vi "Set Group Privilege.vi"(4 "New Value":bool, 5 "Save File":bool=TRUE, 6 "error in (no error)":errorcluster, 7 "Privilege":string, 8 "Group Name":string, 9 "EasyUserManager in":refnum<class "EasyUserManager.lvclass">) -> (0 "error out":errorcluster, 3 "EasyUserManager out":refnum<class "EasyUserManager.lvclass">)   [LabVIEW 2024, in "EasyUserManager.lvclass"]
doc: "Set <B>Privilege</B> (e.g. Operate.Execute) to the specified <B>New Value</B> for the group called <B>Group Name</B>. \n\nThe boolean input <B>Save File</B> controls whether changes are immediately saved to the users file (Default: True)."
uses:
  EasyUserManager.lvclass
  EasyUserManager.lvclass/EasyUserManager.ctl
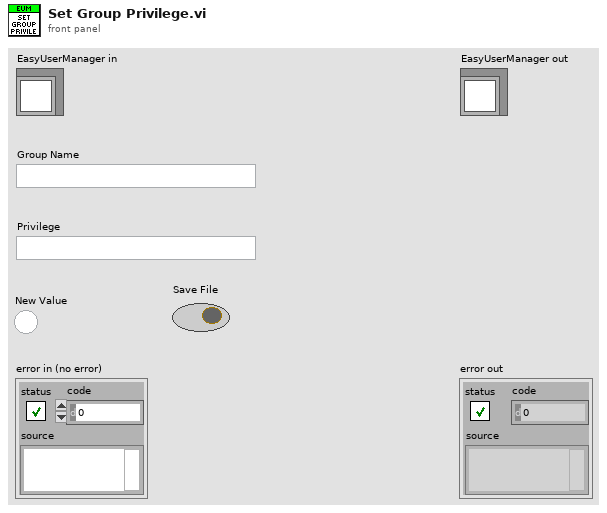
[diagram p1: front panel]
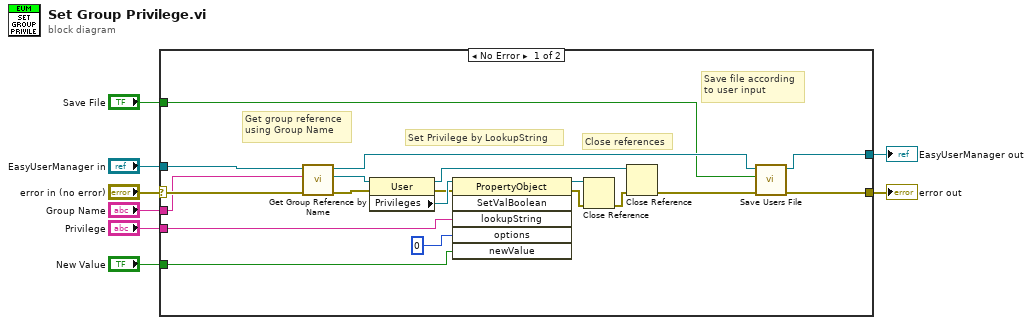
[diagram p0: block diagram]
diagram:
  n1 = case shown="No Error" "error in (no error)" {
    selector: "error in (no error)" -> [w13 w29]
    tunnel: [w14 w29] -> w7
    tunnel: [w16 w28] -> w5
    tunnel: "EasyUserManager in" -> [w27 w28]
    tunnel: "Group Name" -> [w12 _]
    tunnel: "Privilege" -> [w11 _]
    tunnel: "New Value" -> [w10 _]
    tunnel: "Save File" -> [w9 _]
    frame No Error {
      # "Set Privilege by LookupString"
      # "Get group reference\nusing Group Name"
      # "Close references"
      # "Save file according\nto user input"
      n2 = call "Get Group Reference by Name.vi"("error in (no error)"=w13, "Group Name"=w12, "EasyUserManager in"=w27) -> ("error out"=w23:errorcluster, "Group Reference"=w26:refnum<k7>, "EasyUserManager out"=w17:refnum<class "EasyUserManager.lvclass">)  [unwired: 2 in]
      n3 = property on="Property Node" class="User"(reference=w26, error in=w23) -> (reference out=w21:refnum<k7>, error out=w22:errorcluster, "Privileges"=w25:refnum<k7>)
      n4 = invoke on="Invoke Node" class="PropertyObject" method="SetValBoolean"(reference=w25, error in=w22, "lookupString"=w11, "options"=0, "newValue"=w10) -> (reference out=w20:refnum<k7>, error out=w18:errorcluster)  [unwired: 1 in, 4 out]
      n5 = Close Reference(reference=w20, error in (no error)=w18) -> (error out=w19:errorcluster)
      n6 = Close Reference(reference=w21, error in (no error)=w19) -> (error out=w15:errorcluster)
      n7 = call "Save Users File.vi"("error in (no error)"=w15, "Save"=w9, "EasyUserManager in"=w17) -> ("error out"=w14:errorcluster, "EasyUserManager out"=w16:refnum<class "EasyUserManager.lvclass">)  [unwired: 3 in]
    }
    frame Error {
      # "Pass error and do nothing."
    }
  }
  "error out" <- w7
  "EasyUserManager out" <- w5
